vi "Compare Value to Limits.vi"(9 "Tol(%)":dbl, 10 "Variable Monitored":dbl, 11 "Write to AO":dbl) -> (3 "Boolean":bool)   [LabVIEW 2021]
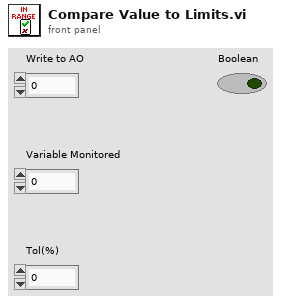
[diagram p1: front panel]
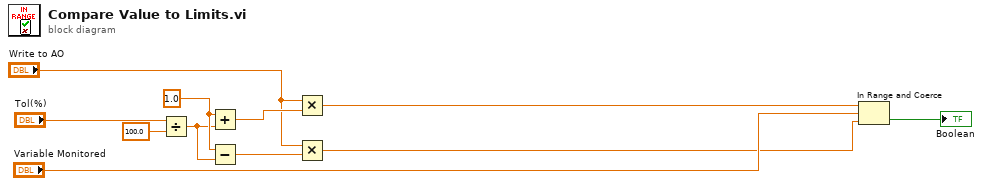
[diagram p0: block diagram]
diagram:
  w5 = 1.0 ("y")
  n1 = Divide(x="Tol(%)", y=100.0) -> (x/y=w4:dbl)
  n2 = Add(x=w5, y=w4) -> (x+y=w7:dbl)
  n3 = Subtract(x=w5, y=w4) -> (x-y=w2:dbl)
  n4 = Multiply(x="Write to AO", y=w7) -> (x*y=w6:dbl)
  n5 = Multiply(x="Write to AO", y=w2) -> (x*y=w1:dbl)
  n6 = In Range and Coerce(upper limit=w6, x="Variable Monitored", lower limit=w1) -> (In Range?=→"Boolean":bool)  [unwired: 1 out]
